vi "to string.vi"(8 "error in":errorcluster, 11 "CVT configuration in":refnum<class "CVT configuration.lvclass">) -> (0 "error out":errorcluster, 1 "data":string, 2 "version":string, 3 "CVT configuration out":refnum<class "CVT configuration.lvclass">)   [LabVIEW 2013, in "CVT configuration.lvclass"]
doc: "Provides an interface for saving a module configuration to a file or other serialized data source. It is recommended that all children of this class store data in two sets--data required for its own initialization, and any data required for parent initialization--and that each implementation uses the <b>Call Parent Method</b> primitive to serialize parent information."
uses:
  CVT configuration.lvclass
  <vilib>/NI/Tag Bus Module Framework/module configuration/TBM module configuration.lvclass
  CVT configuration.lvclass/CVT configuration.ctl
  <vilib>/NI/Configuration Framework/serializable configuration/NISE_CEF_serializable configuration.lvclass
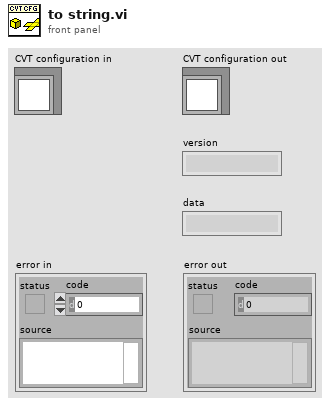
[diagram p1: front panel]
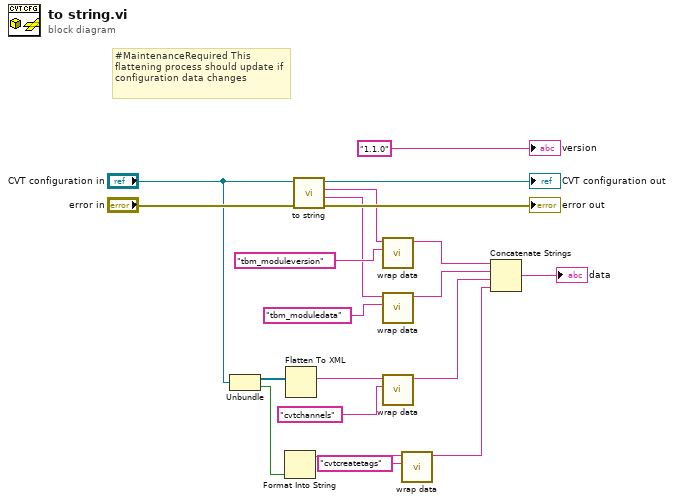
[diagram p0: block diagram]
diagram:
  # "#MaintenanceRequired This flattening process should update if configuration data changes"
  n1 = Unbundle("CVT configuration in") -> (w9:refnum<class "TBM channel.lvclass">[], w3:bool)
  n2 = Format Into String(w3) -> (resulting string=w2:string)  [unwired: 3 in, 1 out]
  n3 = Flatten To XML(anything=w9) -> (xml string=w8:string)
  n4 = call-parent "to string.vi"("error in"="error in", "module configuration in"="CVT configuration in") -> ("error out"=→"error out":errorcluster, "data"=w12:string, "version"=w13:string, "module configuration out"=→"CVT configuration out":refnum<class "CVT configuration.lvclass">)  [unwired: 6 in]
  n5 = call <vilib>:"wrap data.vi"("identifier"="tbm_moduleversion" ("additional identifier"), "data to wrap"=w13) -> ("wrapped data"=w15:string)  [unwired: 9 in]
  n6 = call <vilib>:"wrap data.vi"("identifier"="tbm_moduledata" ("additional identifier"), "data to wrap"=w12) -> ("wrapped data"=w14:string)  [unwired: 9 in]
  n7 = call <vilib>:"wrap data.vi"("identifier"="cvtchannels" ("additional identifier"), "data to wrap"=w8) -> ("wrapped data"=w7:string)  [unwired: 9 in]
  n8 = call <vilib>:"wrap data.vi"("identifier"="cvtcreatetags", "data to wrap"=w2) -> ("wrapped data"=w1:string)  [unwired: 9 in]
  n9 = Concatenate Strings(w15, w14, w7, w1) -> (→"data":string)
  "version" <- "1.1.0" ("current version")
